vi "PicoScope6000ExampleRapidBlock.vi"() -> ()   [LabVIEW 2009]
panel:
  out "Analog Channels":T1(graph)
  out "Device Info":T2
  in  "Channel A Settings":T3 {"Bandwidth" items=["Full", "20 MHz"]; "Range" items=["10 mV", "20 mV", "50 mV", "100 mV", "200 mV", "500 mV", "1 V", "2 V", "5 V", "10 V", "20 V", "50 V ", "100 V"]; "Coupling" items=["AC", "DC 1 MOhm", "DC 50 Ohm"]}
  out "Properties Panel":T4 {"Max Total Capture Time Available (sec)" format="%.3p"; "Sample Frequency" format="%.3p"; "Sample Internal" format="%.3p"; "Max Samples Available" format="%.3p"; "Total Capture Time (sec)" format="%.3p"}
  out "Trigger Offsets":cluster{u64, sgl}[](array[cluster]) {"?" format="%#_5p"}
  out "Trigger Info":T5(array[cluster])
  in  "Rapid Block Acquisition Settings":T6
  in  "Trigger Settings":T7 {"Trigger Direction" items=["Rising", "Falling"]}
  out "Capture Complete":bool
  in  "Run":bool
  in  "Capture Index":i16 min=0
  in  "stop":bool
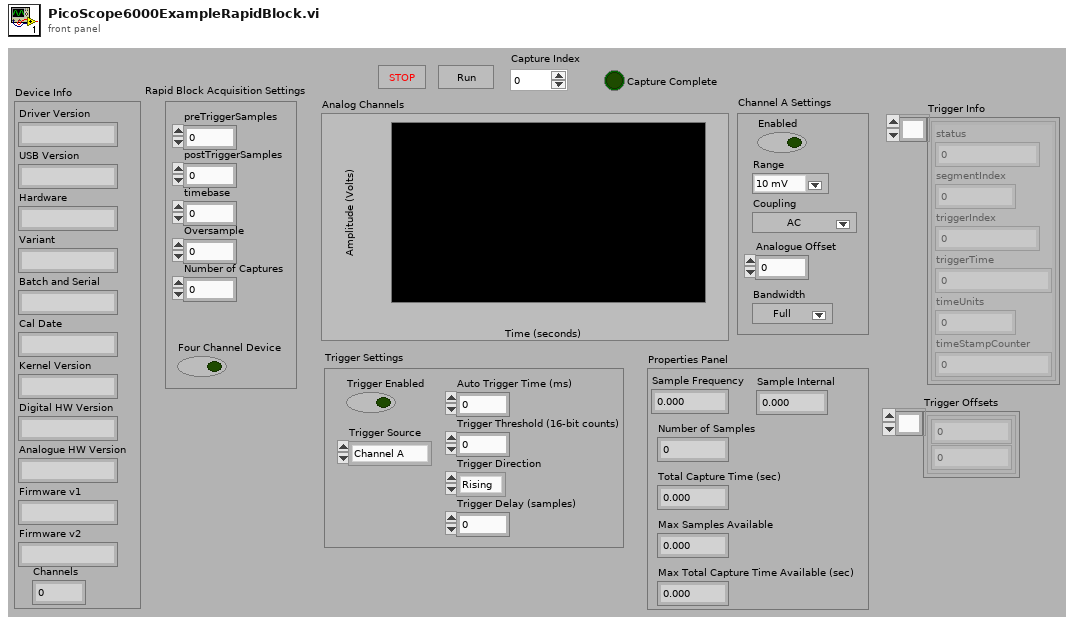
[diagram p1: front panel]
types:
  T1 = cluster{i32, "Sample Internal":sgl, "Data":dbl[]}[]
  T2 = cluster{"Driver Version":string, "USB Version":string, "Hardware":string, "Variant":string, "Batch and Serial":string, "Cal Date":string, "Kernel Version":string, "Digital HW Version":string, "Analogue HW Version":string, "Firmware v1":string, "Firmware v2":string, "Channels":i16}
  T3 = cluster{"Enabled":bool, "Coupling":u32, "Range":u32, "Analogue Offset":sgl, "Bandwidth":u32}
  T4 = cluster{"Sample Frequency":sgl, "Sample Internal":sgl, "maxSamples":u32, "Number of Samples":u32, "Total Capture Time (sec) ":sgl, "Max Total Capture Time Available (sec)":sgl}
  T5 = cluster{"status":u32, "segmentIndex":u32, "triggerIndex":u32, "triggerTime":i64, "timeUnits":i16, "timeStampCounter":u64}[]
  T6 = cluster{"preTriggerSamples":u32, "postTriggerSamples":u32, "timebase":u32, "Four Channel Device":bool, "Oversample":i16, "Number of Captures":u32}
  T7 = cluster{"Trigger Enabled":bool, "Trigger Source":enum32{"Channel A", "Channel B", "Channel C", "Channel D", "External", "Aux."}, "Trigger Threshold (16-bit counts)":i16, "Trigger Direction":u16, "Trigger Delay (samples)":u32, "Auto Trigger Time (ms)":i16}
  T8 = cluster{"Enabled":bool, "Coupling":i32, "Range":u16, "Analogue Offset":sgl, "Bandwidth":i32}
  T9 = cluster{i32, "Sample Internal":sgl, "Data":dbl[]}
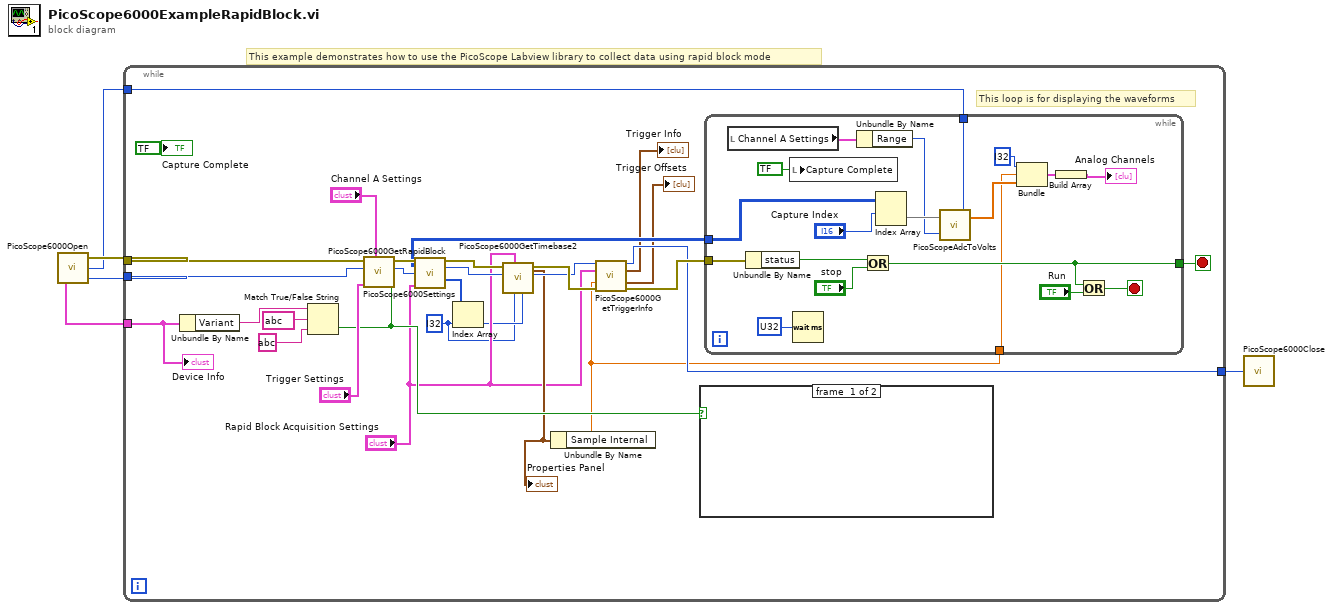
[diagram p0: block diagram]
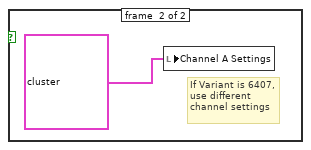
[diagram p2: hidden frame]
diagram:
  # "This example demonstrates how to use the PicoScope Labview library to collect data using rapid block mode"
  n1 = call "PicoScope6000Open.vi"() -> ("handle"=w4:i16, "Max Adc value"=w1:i16, "error out"=w5:errorcluster, "Device Info"=w2:T2)  [unwired: 3 in]
  n2 = while {
    tunnel: w4 -> [w10]
    tunnel: w5 -> [w11]
    tunnel: [w24] -> w3
    tunnel: w2 -> [w9]
    tunnel: w1 -> [w7]
    stop <- w34 stop-if-true
    w13 = i32 ? ("index")
    # "This loop is for displaying the waveforms"
    n3 = Unbundle By Name(w9) -> ("Variant"=w8:string)
    n4 = Match True/False String(2:string ? ("false string"), 3:string ? ("true string"), 4:w8) -> (0:w26:bool)  [unwired: 1 out]
    n5 = call "PicoScope6000Settings.vi"("PS6407?"=w26, "Channel A Settings"="Channel A Settings", "Trigger Settings"="Trigger Settings", "handle in"=w10, "error in"=w11) -> ("handle out"=w30:i16, "error out"=w31:errorcluster)  [unwired: 4 in, 1 out]
    n6 = call "PicoScope6000GetRapidBlock.vi"("error in"=w31, "handle in"=w30, "Rapid Block Acquisition Settings"="Rapid Block Acquisition Settings") -> ("Channel A Buffer"=w29:i16[][], "error out"=w21:errorcluster, "handle out"=w20:i16, "noOfSamples"=w15:u32[])  [unwired: 6 in, 3 out]
    n7 = Index Array(array=w15, index=w13) -> (element=w14:u32)
    n8 = call "PicoScope6000GetTimebase2.vi"("Number of Samples"=w14, "Memory Segment"=w13, "Acquisition Settings"="Rapid Block Acquisition Settings", "handle in"=w20, "error in (no error)"=w21) -> ("handle out"=w18:i16, "error out"=w19:errorcluster, "Properties Panel"=w17:T4)  [unwired: 4 in]
    "Properties Panel" <- w17
    n9 = Unbundle By Name(w17) -> ("Sample Internal"=w6:sgl)
    n10 = call "PicoScope6000GetTriggerInfo.vi"("handle in"=w18, "Rapid Block Acquisition Settings"="Rapid Block Acquisition Settings", "Sample Rate"=w6, "error in"=w19) -> ("handle out"=w24:i16, "Trigger Info"=→"Trigger Info":T5, "Trigger Offsets"=→"Trigger Offsets":cluster{u64, sgl}[], "error out"=w25:errorcluster)  [unwired: 8 in]
    n11 = case shown="True" w26 {
      frame #0 {
      }
      frame #1 {
        # "If Variant is 6407,\nuse different \nchannel settings"
        n12 = local write "Channel A Settings"(T8 ? ("Channel A Settings")) -> ()
      }
    }
    n13 = while {
      tunnel: [w53] -> w34
      tunnel: w29 -> [w46]
      tunnel: w25 -> [w48]
      tunnel: w7 -> [w39]
      tunnel: w6 -> [w36]
      stop <- w52 stop-if-true
      n14 = local read "Channel A Settings"() -> (w38:T3)
      n15 = Unbundle By Name(w48) -> ("status"=w47:bool)
      n16 = local write "Capture Complete"(bool ? ("Capture Complete")) -> ()
      n17 = Wait (ms)(milliseconds to wait=u32 ?) -> ()  [unwired: 1 out]
      n18 = Unbundle By Name(w38) -> ("Range"=w37:u32)
      n19 = Or(x=w47, y="stop") -> (x .or. y?=w53:bool)
      n20 = Index Array(array=w46, index (row)="Capture Index") -> (element=w44:i16[])  [unwired: 1 in]
      n21 = call "PicoScopeAdcToVolts.vi"("Max_adc"=w39, "Range Index"=w37, "Data"=w44) -> ("Data"=w40:dbl[])
      n22 = Bundle(i32 ?, "Sample Internal"=w36, "Data"=w40) -> (w41:T9)  [unwired: 1 in]
      n23 = Build Array(w41) -> (→"Analog Channels":T1)
      n24 = Or(x=w53, y="Run") -> (x .or. y?=w52:bool)
    }
    "Capture Complete" <- bool ? ("Capture Complete")
    "Device Info" <- w9
  }
  n25 = call "PicoScope6000Close.vi"("handle"=w3) -> ()
